vi "Read Server Internal UEs.vi"(8 "error in (no error)":errorcluster, 11 "gRPC service in":refnum<class "CanReaderNixnet.lvclass">) -> (0 "error out":errorcluster, 2 "Server Internal UEs":T1, 3 "gRPC service out":refnum<class "CanReaderNixnet.lvclass">)   [LabVIEW 2021, in "CanReaderNixnet_server.lvlib" / "CanReaderNixnet.lvclass"]
uses:
  CanReaderNixnet.lvclass
  typeDefs/Server Internal UEs.ctl
  typeDefs/Server Internal Message.ctl
  CanReaderNixnet.lvclass/CanReaderNixnet.ctl
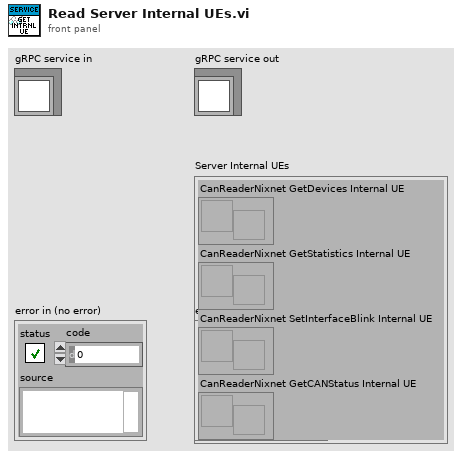
[diagram p1: front panel]
types:
  T1 = typedef "CanReaderNixnet_server.lvlib/CanReaderNixnet.lvclass/Server Internal UEs.ctl" = cluster{"CanReaderNixnet GetDevices Internal UE":refnum<user-event>, "CanReaderNixnet GetStatistics Internal UE":refnum<user-event>, "CanReaderNixnet SetInterfaceBlink Internal UE":refnum<user-event>, "CanReaderNixnet GetCANStatus Internal UE":refnum<user-event>}
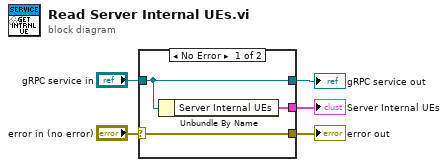
[diagram p0: block diagram]
diagram:
  n1 = case shown="No Error" "error in (no error)" {
    selector: "error in (no error)" -> [w8 w9]
    tunnel: [w8 w9] -> w4
    tunnel: [w7 w10] -> w2
    tunnel: "gRPC service in" -> [w7 w10]
    tunnel: [w6 _] -> w1
    frame No Error {
      n2 = Unbundle By Name(w7) -> ("Server Internal UEs"=w6:T1)
    }
    frame Error {
    }
  }
  "error out" <- w4
  "gRPC service out" <- w2
  "Server Internal UEs" <- w1
